vi "system_config.vi"() -> ()   [LabVIEW 2026]
uses:
  <vilib>/addons/_JKI.lib/Serialization/JSON/JKI JSON Serialization.lvlib
panel:
  in  "Cluster":T1
  out "Preview":string
  in  "Number of Node":i32
  in  "Array":T2(array[cluster])
  in  "Clear / Reset":bool
  in  "Generate JSON":bool
  in  "?":bool
  out "Node Count":dbl
  out "Status Message":string
  in  "Save Path":path
  # "Scenario Global Settings"
  # "Actions"
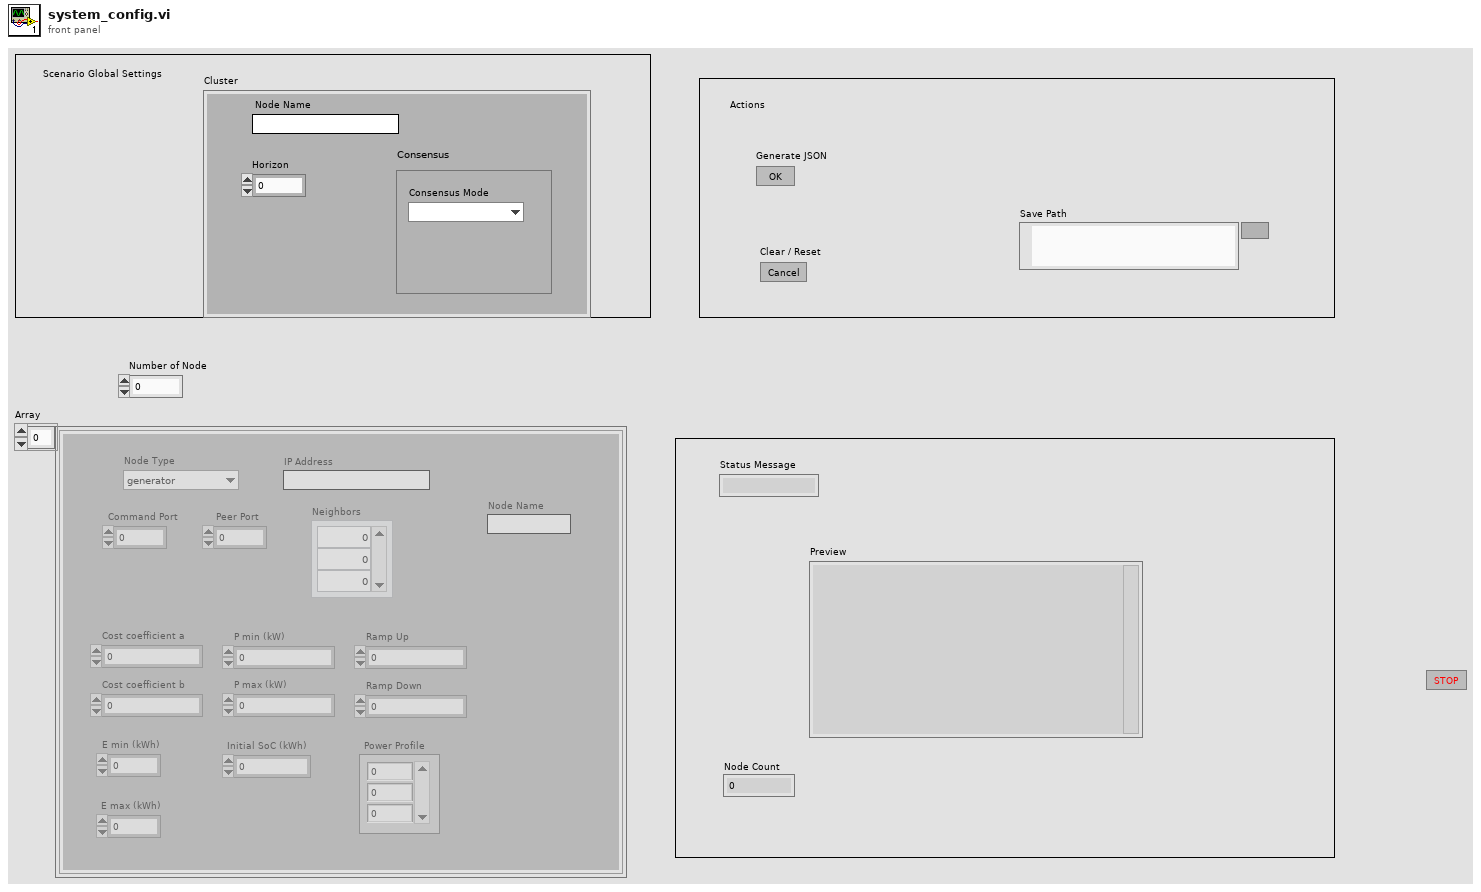
[diagram p1: front panel]
types:
  T1 = cluster{"horizon":i32, "name":string, "consensus":cluster{"consensus.mode":u16}}
  T2 = cluster{"name":string, "IP Address":string, "Command Port":dbl, "Peer Port":dbl, "Neighbors":dbl[], "a":dbl, "b":dbl, "p_min":dbl, "p_max":dbl, "ramp_up":dbl, "ramp_down":dbl, "e_min":dbl, "e_max":dbl, "e_init":dbl, "profile":dbl[], "type":enum16{"generator", "load", "battery"}}[]
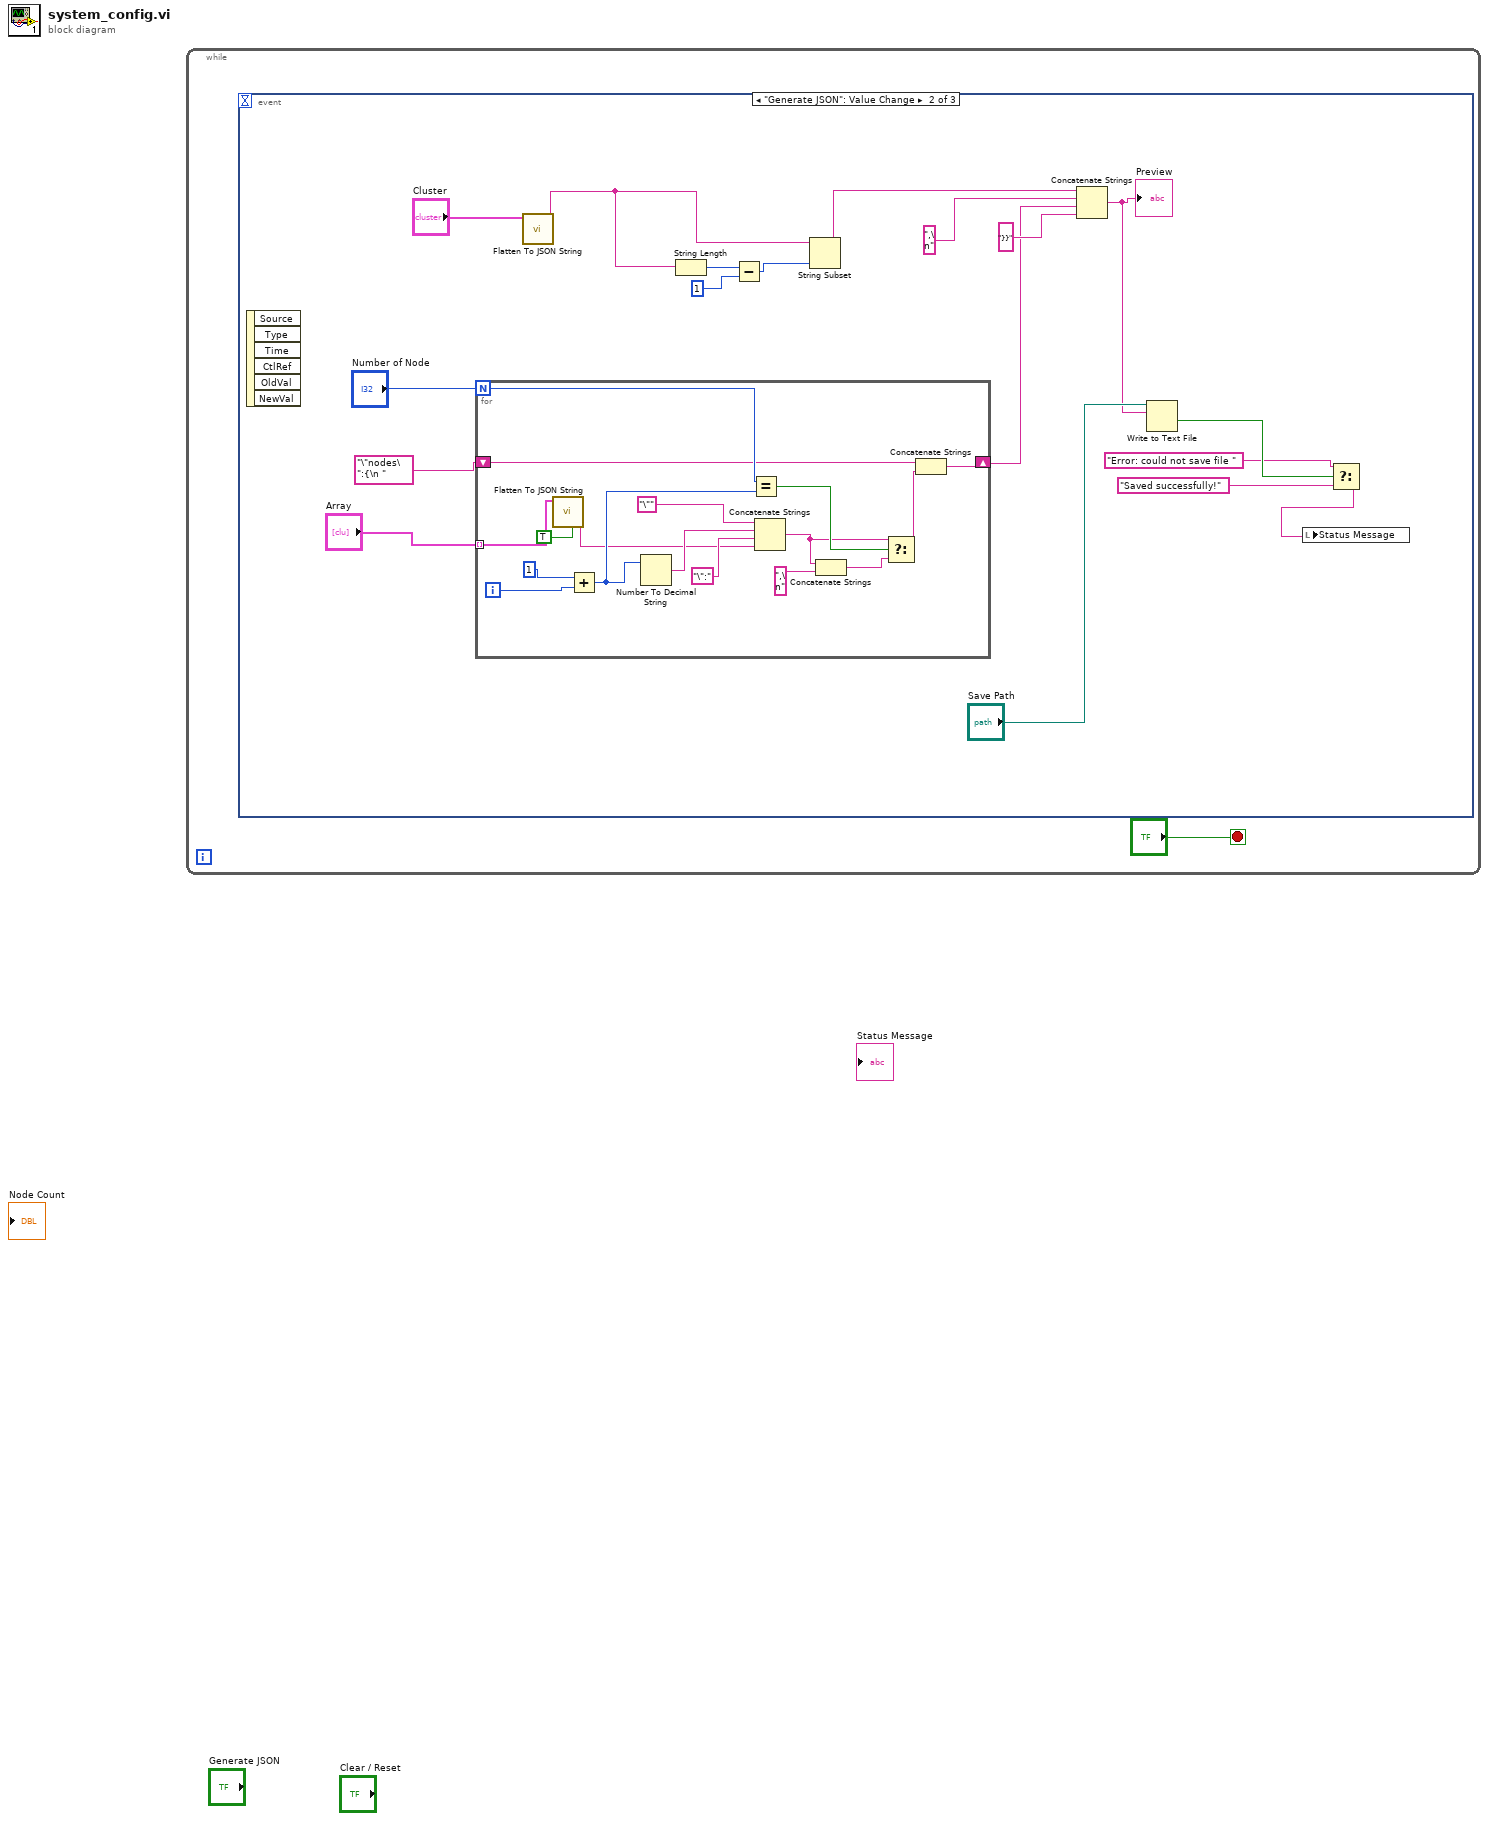
[diagram p0: block diagram]
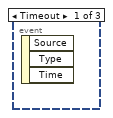
[diagram p2: hidden frame]
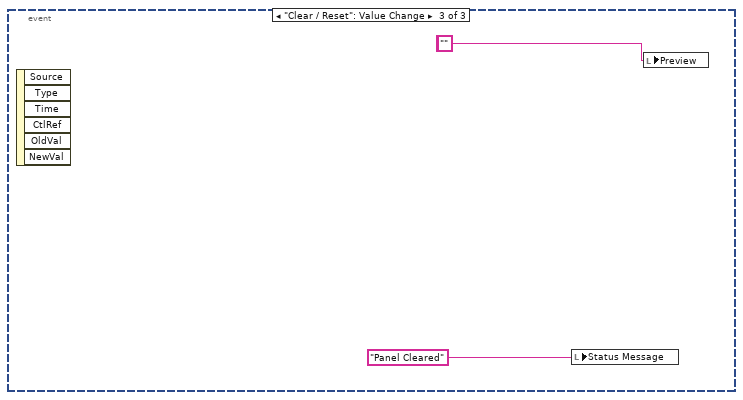
[diagram p3: hidden frame]
diagram:
  n1 = while {
    stop <- "?" stop-if-true
    n2 = event shown="[1] \"Generate JSON\": Value Change" {
      selector: _ -> [_ _ _]
      dyn-events: _ -> [_ _ _]
      timeout: _ -> [_ _ _]
      event Timeout {
        n3 = event-data() -> ()  [unwired: 1 in, 3 out]
      }
      event "Generate JSON": Value Change {
        n4 = event-data() -> ()  [unwired: 1 in, 6 out]
        n5 = for {
          N: "Number of Node" -> [w32]
          tunnel: "Array" -> [w24] mode=indexing
          shift-right: [w25] -> w9
          shift-left: "\"nodes\":{\n " -> [w27]
          i -> [w36]
          n6 = call <vilib>:"Flatten To JSON String.vi"("Enums As String (F)"=TRUE, "Variant"=w24) -> ("JSON String"=w21:string)  [unwired: 8 in, 1 out]
          n7 = Add(x=1, y=w36) -> (x+y=w33:i32)
          n8 = Number To Decimal String(number=w33) -> (decimal integer string=w23:string)  [unwired: 1 in]
          n9 = Equal?(x=w32, y=w33) -> (x = y?=w30:bool)
          n10 = Concatenate Strings("\"", w23, "\":", w21) -> (w29:string)
          n11 = Concatenate Strings(w29, ",\n") -> (w28:string)
          n12 = Select(t=w29, s=w30, f=w28) -> (s? t:f=w26:string)
          n13 = Concatenate Strings(w27, w26) -> (w25:string)
        }
        n14 = call <vilib>:"Flatten To JSON String.vi"("Variant"="Cluster") -> ("JSON String"=w13:string)  [unwired: 9 in, 1 out]
        n15 = String Length(string=w13) -> (length=w12:i32)
        n16 = Subtract(x=w12, y=1) -> (x-y=w10:i32)
        n17 = String Subset(string=w13, length (rest)=w10) -> (substring=w14:string)  [unwired: 1 in]
        n18 = Concatenate Strings(w14, ",\n", w9, "}}") -> (w6:string)
        "Preview" <- w6
        n19 = Write to Text File(file (use dialog)="Save Path", text=w6) -> (cancelled=w5:bool)  [unwired: 2 in, 2 out]
        n20 = Select(t="Error: could not save file ", s=w5, f="Saved successfully!") -> (s? t:f=w2:string)
        n21 = local write "Status Message"(w2) -> ()
      }
      event "Clear / Reset": Value Change {
        (unwired) ""
        n22 = event-data() -> ()  [unwired: 1 in, 6 out]
        n23 = local write "Status Message"("Panel Cleared") -> ()
        n24 = local write "Preview"("") -> ()
      }
    }
  }
